vi "VIH Utility - FILE - Relative Path to Absolute Path.vi"(7 "base path (empty: dir of Top VI)":path, 8 "error in":errorcluster, 11 "Path":path) -> (0 "error out":errorcluster, 3 "Path out":path)   [LabVIEW 2014]
doc: "::: VI Helpeks :::\nCopyright (c) 2000-2026 Konstantin Shifershteyn. All rights reserved."
panel:
  # "VI Helpeks\nCopyright (c) 2012-2026 Konstantin Shifershteyn"
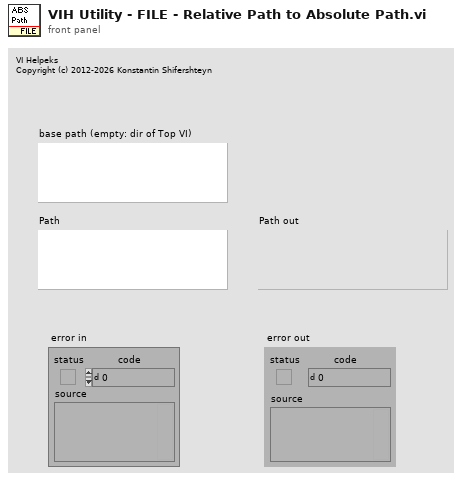
[diagram p1: front panel]
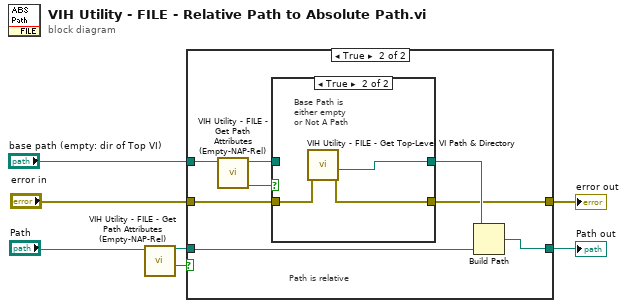
[diagram p0: block diagram]
diagram:
  n1 = call "VIH Utility - FILE - Get Path Attributes (Empty-NAP-Rel).vi"("Path"="Path") -> ("Relative path"=w1:bool, "dup Path"=w3:path)  [unwired: 9 out]
  n2 = case shown="True" w1 {
    tunnel: w3 -> [w9 w17]
    tunnel: [w9 w15] -> w7
    tunnel: "base path (empty: dir of Top VI)" -> [_ w12]
    tunnel: "error in" -> [w8 w14]
    tunnel: [w8 w13] -> w4
    frame False {
    }
    frame True {
      # "Path is relative"
      n3 = call "VIH Utility - FILE - Get Path Attributes (Empty-NAP-Rel).vi"("Path"=w12) -> ("Not A Path or Empty path"=w10:bool, "dup Path"=w11:path)  [unwired: 9 out]
      n4 = case shown="True" w10 {
        tunnel: [w19 w20] -> w16
        tunnel: w11 -> [w19 _]
        tunnel: w14 -> [w18 w22]
        tunnel: [w18 w21] -> w13
        frame False {
        }
        frame True {
          # "Base Path is\neither empty\nor Not A Path"
          n5 = call "VIH Utility - FILE - Get Top-Level VI Path & Directory.vi"("error in"=w22) -> ("error out"=w21:errorcluster, "VI Directory out of .LLB"=w20:path)  [unwired: 9 out]
        }
      }
      n6 = Build Path(base path=w16, name or relative path=w17) -> (appended path=w15:path)
    }
  }
  "Path out" <- w7
  "error out" <- w4
